vi "lvmcp_srright.vi"() -> ()   [LabVIEW 2015]
panel:
  out "error out":errorcluster
  out "top":i32
  out "UID":i32
  in  "reference":refnum<vi>
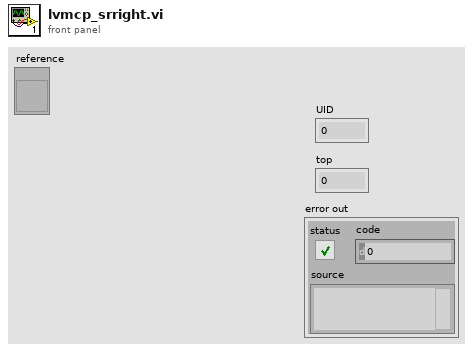
[diagram p1: front panel]
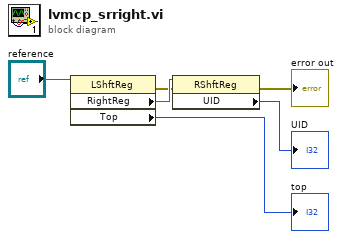
[diagram p0: block diagram]
diagram:
  n1 = property class="LShftReg"(reference="reference") -> (error out=w4:errorcluster, "RightReg"=w5:refnum<vi>, "Top"=→"top":i32)  [unwired: 1 in, 1 out]
  n2 = property class="RShftReg"(reference=w5, error in=w4) -> (error out=→"error out":errorcluster, "UID"=→"UID":i32)  [unwired: 1 out]
